vi "App Run.vi"(8 "error in (no error)":errorcluster, 10 "Core APIs":T1, 11 "DemoApp in":refnum<class "DemoApp.lvclass">) -> (0 "error out":errorcluster)   [LabVIEW 2020, in "VolatusDemo.lvlib" / "DemoApp.lvclass"]
uses:
  DemoApp.lvclass
  Volatus/Core APIs.ctl
  Volatus/VolatusAPI/VolatusAPI.lvclass
  DemoApp.lvclass/DemoApp.ctl
  Volatus/Volatus.lvlib
panel:
  in  "Stop Log":bool
  in  "Start Log":bool
  in  "Test Series":string
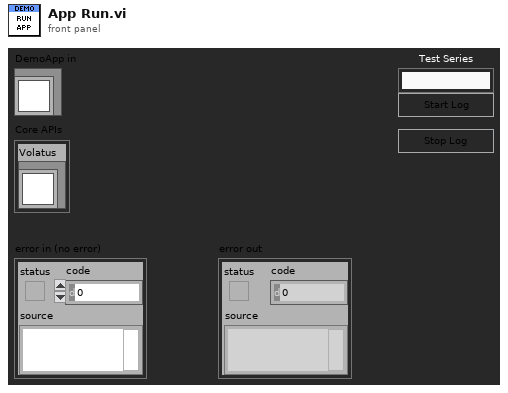
[diagram p1: front panel]
types:
  T1 = typedef "Volatus.lvlib/Core APIs.ctl" = cluster{"Volatus":refnum<class "VolatusAPI.lvclass">}
  T2 = enum8{"Enabled", "Disabled", "Disabled and Grayed Out"}
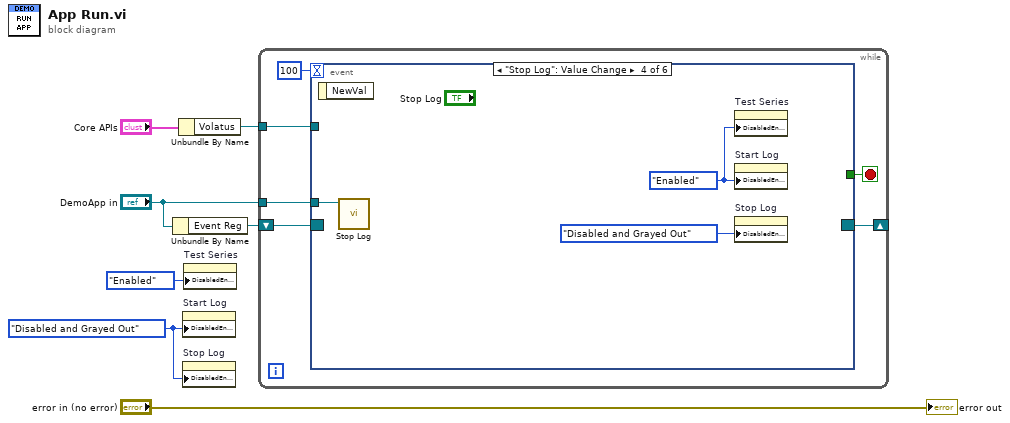
[diagram p0: block diagram]
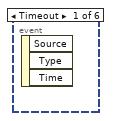
[diagram p2: hidden frame]
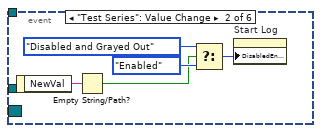
[diagram p3: hidden frame]
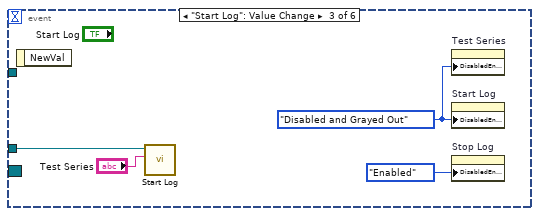
[diagram p4: hidden frame]
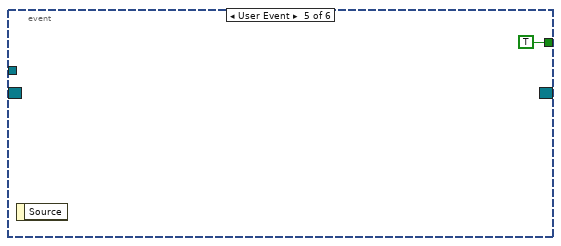
[diagram p5: hidden frame]
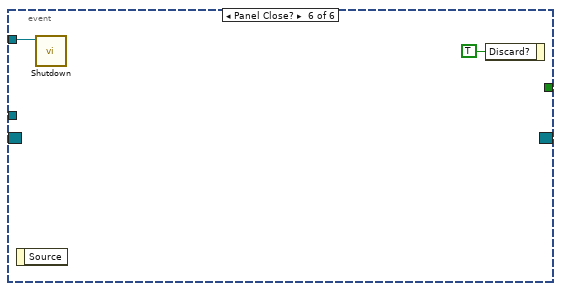
[diagram p6: hidden frame]
diagram:
  w3 = T2."Disabled and Grayed Out" ("Disabled")
  n1 = Unbundle By Name("DemoApp in") -> ("Event Reg"=w6:refnum<event-registration>)
  n2 = Unbundle By Name("Core APIs") -> ("Volatus"=w5:refnum<class "VolatusAPI.lvclass">)
  n3 = property on="Start Log" class="Bool"("DisabledEnum"=w3) -> ()  [unwired: 2 in, 2 out]
  n4 = property on="Stop Log" class="Bool"("DisabledEnum"=w3) -> ()  [unwired: 2 in, 2 out]
  n5 = property on="Test Series" class="Str"("DisabledEnum"=T2."Enabled" ("Disabled")) -> ()  [unwired: 2 in, 2 out]
  n6 = while {
    shift-right: [w11] -> _
    shift-left: w6 -> [w12]
    tunnel: w5 -> [w10]
    tunnel: "DemoApp in" -> [w8]
    stop <- w9 stop-if-true
    n7 = event shown="[3] \"Stop Log\": Value Change" {
      selector: w12 -> [_ _ _ _ _ _]
      dyn-events: [_ _ _ _ _ _] -> w11
      timeout: 100 -> [_ _ _ _ _ _]
      tunnel: w10 -> [_ _ _ _ _ w27]
      tunnel: [_ _ _ _ TRUE _] -> w9
      tunnel: w8 -> [_ _ w21 w25 _ _]
      event Timeout {
        n8 = event-data() -> ()  [unwired: 1 in, 3 out]
      }
      event "Test Series": Value Change {
        n9 = event-data() -> ("NewVal"=w18:string)  [unwired: 1 in]
        n10 = Empty String/Path?(string/path=w18) -> (empty?=w15:bool)
        n11 = Select(t=T2."Disabled and Grayed Out" ("Disabled"), s=w15, f=T2."Enabled") -> (s? t:f=w14:T2)
        n12 = property on="Start Log" class="Bool"("DisabledEnum"=w14) -> ()  [unwired: 2 in, 2 out]
      }
      event "Start Log": Value Change {
        w19 = T2."Disabled and Grayed Out" ("Disabled")
        n13 = event-data() -> ()  [unwired: 1 in, 1 out]
        n14 = call "Start Log.vi"("Test Series"="Test Series", "DemoApp in"=w21) -> ()  [unwired: 8 in, 2 out]
        n15 = property on="Test Series" class="Str"("DisabledEnum"=w19) -> ()  [unwired: 2 in, 2 out]
        n16 = property on="Start Log" class="Bool"("DisabledEnum"=w19) -> ()  [unwired: 2 in, 2 out]
        n17 = property on="Stop Log" class="Bool"("DisabledEnum"=T2."Enabled" ("Disabled")) -> ()  [unwired: 2 in, 2 out]
      }
      event "Stop Log": Value Change {
        w24 = T2."Enabled" ("Disabled")
        n18 = event-data() -> ()  [unwired: 1 in, 1 out]
        n19 = call "Stop Log.vi"("DemoApp in"=w25) -> ()  [unwired: 9 in, 2 out]
        n20 = property on="Test Series" class="Str"("DisabledEnum"=w24) -> ()  [unwired: 2 in, 2 out]
        n21 = property on="Start Log" class="Bool"("DisabledEnum"=w24) -> ()  [unwired: 2 in, 2 out]
        n22 = property on="Stop Log" class="Bool"("DisabledEnum"=T2."Disabled and Grayed Out" ("Disabled")) -> ()  [unwired: 2 in, 2 out]
      }
      event User Event {
        n23 = event-data() -> ()  [unwired: 1 in, 1 out]
      }
      event Panel Close? {
        n24 = event-data() -> ()  [unwired: 1 in, 1 out]
        n25 = call "Shutdown.vi"("VolatusAPI in"=w27) -> ()  [unwired: 9 in, 2 out]
        n26 = event-data("Discard?"=TRUE) -> ()  [unwired: 1 in, 1 out]
      }
    }
  }
  "error out" <- "error in (no error)"
